vi "Write to Data Source.vi"(7 "Project Store in":refnum<class "Project Store-INI.lvclass">, 8 "error in (no error)":errorcluster) -> (0 "error out":errorcluster, 5 "Project Store out":refnum<class "Project Store-INI.lvclass">)   [LabVIEW 2024, in "Project Store-INI.lvclass"]
doc: "Writes the in-memory projects to Projects.ini and the tasks to Tasks.ini in the data folder, each a FULL REWRITE: the old file is replaced, so removed rows disappear. Projects are written in Sort Order; tasks are grouped by project in the same order and then by their own Sort Order, each carrying its project name as the Project Name label. A task whose project no longer exists is still written, last, with an empty label.\n\nGenerated by: Claude"
uses:
  Project Store-INI.lvclass
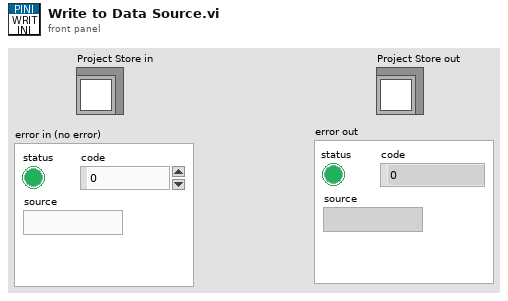
[diagram p1: front panel]
types:
  T1 = typedef "Project List.ctl" = T2[]
  T2 = typedef "Project.ctl" = cluster{"ID":string, "Name":string, "Active":bool, "Sort Order":i32}
  T3 = typedef "Task List.ctl" = T4[]
  T4 = typedef "Task.ctl" = cluster{"ID":string, "Project ID":string, "Name":string, "Active":bool, "Sort Order":i32}
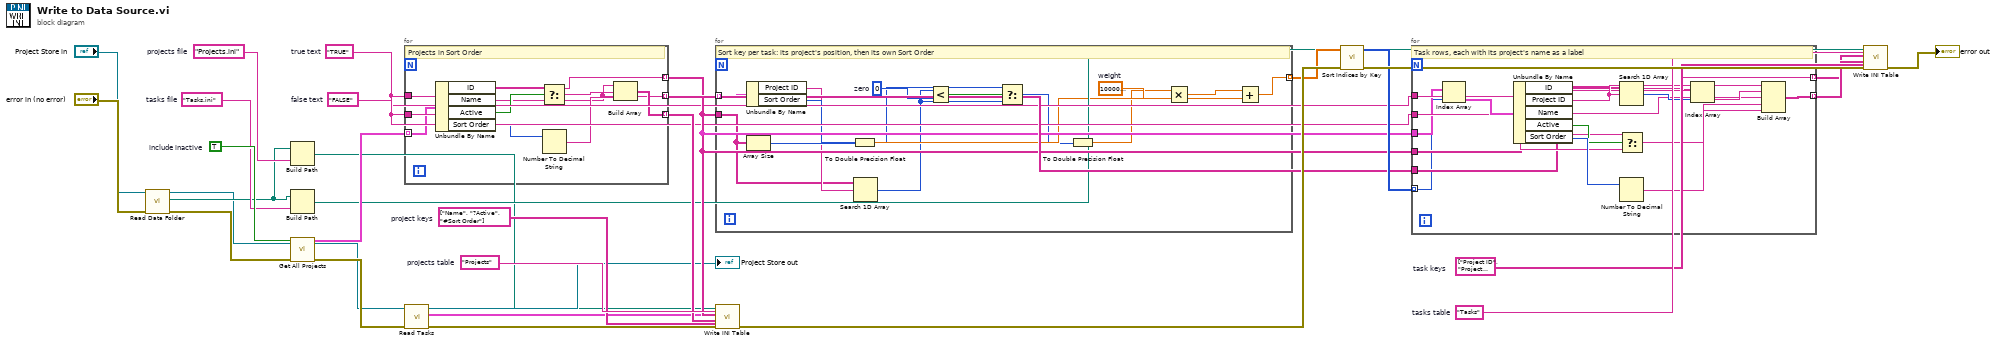
[diagram p0: block diagram]
diagram:
  w29 = "Tasks"  # tasks table
  w28 = "Projects"  # projects table
  w27 = string[] ["Project ID", "Project Name", "Name", "?Active", "#Sort Order"]  # task keys
  w26 = string[] ["Name", "?Active", "#Sort Order"]  # project keys
  w18 = "FALSE"  # false text
  w17 = "TRUE"  # true text
  w10 = TRUE  # include inactive
  w7 = "Tasks.ini"  # tasks file
  w6 = "Projects.ini"  # projects file
  n1 = call-dynamic "Read Data Folder.vi"("error in (no error)"="error in (no error)", "Project Store-INI in"="Project Store in") -> ("error out"=w3:errorcluster, "Data Folder"=w5:path, "Project Store-INI out"=w4:refnum<class "Project Store-INI.lvclass">)  [unwired: 7 in]
  n2 = Build Path(base path=w5, name or relative path=w6) -> (appended path=w8:path)
  n3 = Build Path(base path=w5, name or relative path=w7) -> (appended path=w9:path)
  n4 = call-dynamic "Get All Projects.vi"("Project Store in"=w4, "error in (no error)"=w3, "include inactive?"=w10) -> ("error out"=w13:errorcluster, "Projects"=w12:T1, "Project Store out"=w11:refnum<class "Project Store-INI.lvclass">)  [unwired: 6 in]
  n5 = for {
    tunnel: w17 -> [w33]
    tunnel: w18 -> [w34]
    tunnel: w12 -> [w32] mode=indexing
    tunnel: [w35] -> w19 mode=indexing
    tunnel: [w36] -> w21 mode=indexing
    tunnel: [w41] -> w20 mode=indexing
    # "Projects in Sort Order"
    n6 = Unbundle By Name(w32) -> ("ID"=w35:string, "Name"=w36:string, "Active"=w37:bool, "Sort Order"=w38:i32)
    n7 = Select(t=w33, s=w37, f=w34) -> (s? t:f=w39:string)
    n8 = Number To Decimal String(number=w38) -> (decimal integer string=w40:string)  [unwired: 1 in]
    n9 = Build Array(w36, w39, w40) -> (w41:string[])
  }
  n10 = call-dynamic "Read Tasks.vi"("error in (no error)"=w13, "Project Store in"=w11) -> ("error out"=w14:errorcluster, "Task List"=w16:T3, "Project Store out"=→"Project Store out":refnum<class "Project Store-INI.lvclass">)  [unwired: 7 in]
  n11 = for {
    tunnel: w16 -> [w42] mode=indexing
    tunnel: w19 -> [w43]
    tunnel: [w55] -> w22 mode=indexing
    w52 = 1000000.0  # weight
    w48 = 0  # zero
    # "Sort key per task: its project's position, then its own Sort Order"
    n12 = Unbundle By Name(w42) -> ("Project ID"=w44:string, "Sort Order"=w45:i32)
    n13 = Array Size(array=w43) -> (size(s)=w47:i32)
    n14 = To Double Precision Float(number=w45) -> (double precision float=w54:dbl)
    n15 = Search 1D Array(1D array=w43, element=w44) -> (index of element=w46:i32)  [unwired: 1 in]
    n16 = Less?(x=w46, y=w48) -> (x < y?=w49:bool)
    n17 = Select(t=w47, s=w49, f=w46) -> (s? t:f=w50:i32)
    n18 = To Double Precision Float(number=w50) -> (double precision float=w51:dbl)
    n19 = Multiply(x=w51, y=w52) -> (x*y=w53:dbl)
    n20 = Add(x=w53, y=w54) -> (x+y=w55:dbl)
  }
  n21 = call "Write INI Table.vi"("Keys"=w26, "Table Name"=w28, "error in (no error)"=w14, "Values"=w20, "Section Names"=w19, "File Path"=w8) -> ("error out"=w30:errorcluster)  [unwired: 5 in]
  n22 = call "Sort Indices by Key.vi"("Keys"=w22) -> ("Sorted Indices"=w23:i32[])  [unwired: 9 in, 1 out]
  n23 = for {
    tunnel: w17 -> [w60]
    tunnel: w18 -> [w61]
    tunnel: w16 -> [w57]
    tunnel: w19 -> [w58]
    tunnel: w21 -> [w59]
    tunnel: w23 -> [w56] mode=indexing
    tunnel: [w63] -> w24 mode=indexing
    tunnel: [w72] -> w25 mode=indexing
    # "Task rows, each with its project's name as a label"
    n24 = Index Array(array=w57, index=w56) -> (element=w62:T4)
    n25 = Unbundle By Name(w62) -> ("ID"=w63:string, "Project ID"=w64:string, "Name"=w65:string, "Active"=w66:bool, "Sort Order"=w67:i32)
    n26 = Search 1D Array(1D array=w58, element=w64) -> (index of element=w68:i32)  [unwired: 1 in]
    n27 = Select(t=w60, s=w66, f=w61) -> (s? t:f=w70:string)
    n28 = Number To Decimal String(number=w67) -> (decimal integer string=w71:string)  [unwired: 1 in]
    n29 = Index Array(array=w59, index=w68) -> (element=w69:string)
    n30 = Build Array(w64, w69, w65, w70, w71) -> (w72:string[])
  }
  n31 = call "Write INI Table.vi"("Keys"=w27, "Table Name"=w29, "error in (no error)"=w30, "Values"=w25, "Section Names"=w24, "File Path"=w9) -> ("error out"=→"error out":errorcluster)  [unwired: 5 in]
